vi "G4SubTemplate_Singleton_4x4x4_CleanUp.vi"(8 "Error In":errorcluster) -> (0 "Error Out":errorcluster)   [LabVIEW 2020, in "G4SubTemplate_Singleton_4x4x4.lvclass"]
uses:
  G4SubTemplate_Singleton_4x4x4.lvclass
  G4BaseTemplate_Singleton_4x4x4/G4BaseTemplate_Singleton_4x4x4.lvclass
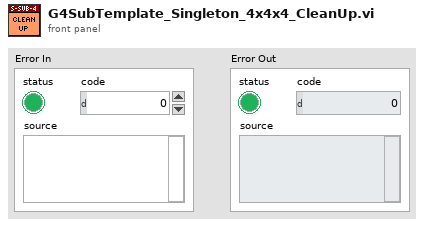
[diagram p1: front panel]
types:
  T1 = typedef "G4SubTemplate_Singleton_4x4x4.lvclass/ObjectAttributes.ctl" = cluster{"Attribute1":dbl}
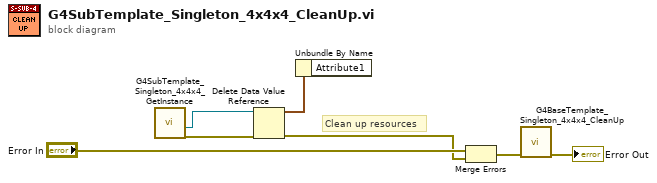
[diagram p0: block diagram]
diagram:
  # "Clean up resources"
  n1 = call "G4SubTemplate_Singleton_4x4x4_GetInstance.vi"() -> ("Error Out"=w2:errorcluster, "DVRRefOut"=w3:refnum<data-value>)  [unwired: 7 in, 3 out]
  n2 = Delete Data Value Reference(data value reference=w3, error in=w2) -> (data value=w1:T1, error out=w4:errorcluster)
  n3 = Unbundle By Name(w1) -> ()  [unwired: 1 out]
  n4 = Merge Errors("Error In", w4) -> (w7:errorcluster)
  n5 = call "G4BaseTemplate_Singleton_4x4x4_CleanUp.vi"("Error In"=w7) -> ("Error Out"=→"Error Out":errorcluster)  [unwired: 10 in]
